vi "Clear Fault.vi"(8 "error in":errorcluster, 9 "timeout (-1)":i32=-1, 10 "code (0=clear all)":i32, 11 "Engine Runtime Interface in":refnum<class "Engine Runtime Interface.lvclass">) -> (0 "error out":errorcluster, 3 "Engine Runtime Interface out":refnum<class "Engine Runtime Interface.lvclass">)   [LabVIEW 2014, in "Engine Runtime Interface.lvclass"]
doc: "Clears the record of a fault in the engine. If the fault selected is code 0, it clears all faults."
uses:
  Engine Runtime Interface.lvclass
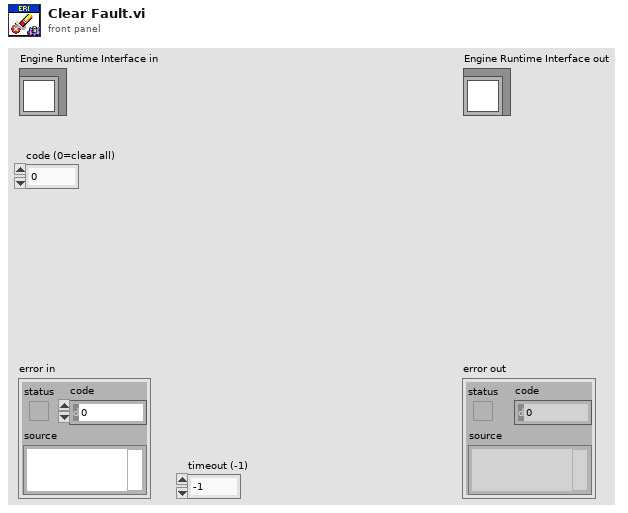
[diagram p1: front panel]
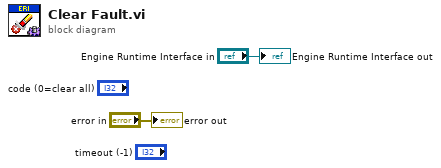
[diagram p0: block diagram]
diagram:
  "error out" <- "error in"
  "Engine Runtime Interface out" <- "Engine Runtime Interface in"
